vi "Convert Multiple.vi"() -> ()   [LabVIEW 2020]
panel:
  in  "Output folder":path
  out "Batch progress":dbl(slide) scale=0.0..1.0
  out "Converting...":path
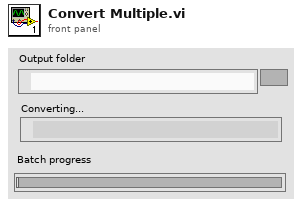
[diagram p1: front panel]
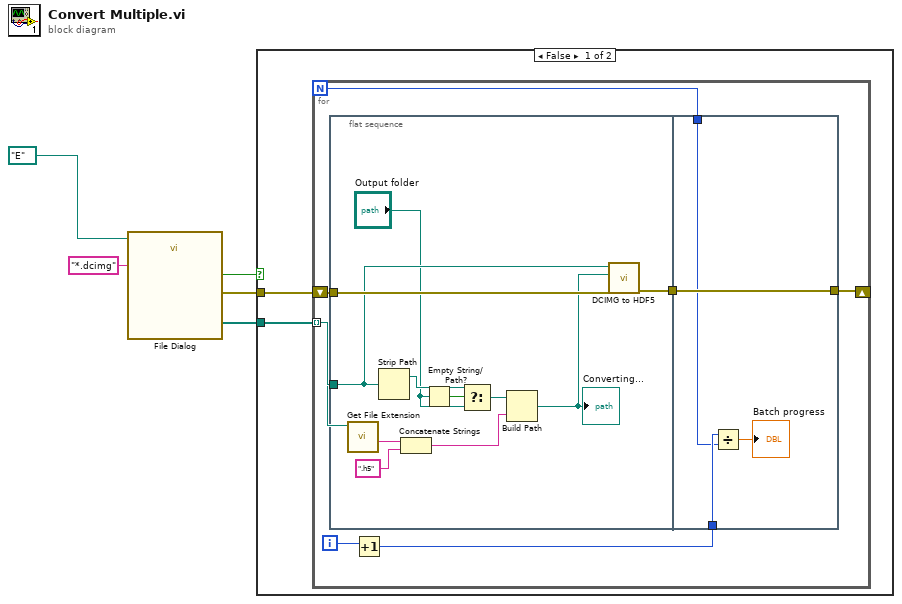
[diagram p0: block diagram]
diagram:
  n1 = call "File Dialog"("start path"=path "E:/", "pattern (all files)"="*.dcimg") -> ("selected paths"=w1:path[], "cancelled"=w3:bool, "error out"=w2:errorcluster)  [unwired: 10 in, 1 out]
  n2 = case shown="False" w3 {
    tunnel: w2 -> [w6 _]
    tunnel: w1 -> [w7 _]
    frame False {
      n3 = for {
        N -> [w10]
        tunnel: w7 -> [w12] mode=indexing
        shift-right: [w13] -> _
        shift-left: w6 -> [w14]
        i -> [w9]
        n4 = flat-sequence {
          tunnel: w14 -> [w25]
          tunnel: w12 -> [w19]
          tunnel: [w24] -> w11
          tunnel: [w29] -> w13
          tunnel: w11 -> [w29]
          tunnel: w8 -> [w27]
          tunnel: w10 -> [w26]
          frame #0 {
            n5 = call <vilib>:"Get File Extension.vi"("file"=w19) -> ("filename without extension"=w23:string)  [unwired: 6 in, 4 out]
            n6 = Strip Path(path=w19) -> (stripped path=w17:path)  [unwired: 1 out]
            n7 = Concatenate Strings(w23, ".h5" ("string")) -> (w21:string)
            n8 = Empty String/Path?(string/path="Output folder") -> (empty?=w15:bool)
            n9 = Select(t=w17, s=w15, f="Output folder") -> (s? t:f=w18:path)
            n10 = Build Path(base path=w18, name or relative path=w21) -> (appended path=w20:path)
            "Converting..." <- w20
            n11 = call "DCIMG to HDF5.vi"("error in (no error)"=w25, "Output path (*.h5)"=w20, "Input path (*.dcimg)"=w19) -> ("error out"=w24:errorcluster)  [unwired: 8 in]
          }
          frame #1 {
            n12 = Divide(x=w27, y=w26) -> (x/y=→"Batch progress":dbl)
          }
        }
        n13 = Increment(x=w9) -> (x+1=w8:i32)
      }
    }
    frame True {
    }
  }
